vi "var to string (string).vi"(10 "String type":string, 11 "reference":refnum<vi>) -> (3 "string":string)   [LabVIEW 2025]
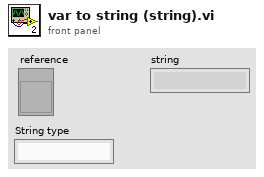
[diagram p1: front panel]
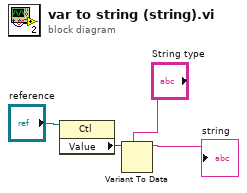
[diagram p0: block diagram]
diagram:
  n1 = property class="Ctl"(reference="reference") -> ("Value"=w4:variant)  [unwired: 1 in, 2 out]
  n2 = Variant To Data(type="String type", Variant=w4) -> (data=→"string":string)  [unwired: 1 in, 1 out]
